vi "Resonance_Test.vi"(0 "Semiconductor Module Context":T7, 1 "FGEN Pin":T1, 2 "SCOPE Pins":T1[](array[typedef]), 3 "FGEN_Parameters":T2 {"Trigger Mode" items=["Single", "Continuous", "Stepped", "Burst"]}, 4 "SCOPE_Parameters":T4={"min sample rate"=20000000.0, "min record length"=1000, "reference position"=5.0, "input impedance"=0, "maximum input frequency"=0.0, "vertical coupling"=1, "vertical range"=10.0, "vertical offset"=0.0, "NumRecords"=0} {"maximum input frequency" format="%.2f"; "input impedance" items=["1 mega ohm"=0, "50 ohms"=2]; "vertical offset" format="%.4f"; "vertical range" format="%.2f"; "vertical coupling" items=["AC", "DC", "Ground"]; "reference position" format="%#_13g"; "min sample rate" format="%^.2e"}, 6 "Published Data Id":T6) -> (19 "error out":errorcluster)   [LabVIEW 2023, in "Resonance.lvlib"]
doc: "Configures SMU/AWG and start generating; if using SMU it also measures back the voltage applied.\nThe SCOPE acquires N channels and averages the samples of each channel.\nThe Offset is computed by dividing the average value with the applied voltage or Vrms of Sine wave when using AWG"
uses:
  Resonance.lvlib
  <vilib>/NI_TestStand_SemiconductorModule/NI_TestStand_Semiconductor_Module.lvlibp/PinMap/General/SemiconductorModuleContext.ctl
  <vilib>/NI_TestStand_SemiconductorModule/NI_TestStand_Semiconductor_Module.lvlibp/PinMap/TagProvider/TSM_Pin.ctl
  <vilib>/NI_TestStand_SemiconductorModule/NI_TestStand_Semiconductor_Module.lvlibp/PinMap/TagProvider/TSM_PublishedDataId.ctl
  ResourceHandling/TypeDefs/RH_SCOPE_Parameters.ctl
  <instrlib>/niScope/Controls/niScope vertical coupling.ctl
  ResourceHandling/TypeDefs/RH_FGEN_Parameters.ctl
  <instrlib>/niFgen/niFgen.llb/niFgen Trigger Mode.ctl
  <instrlib>/niFgen/niFgen.llb/niFgen_ctl Exported Signal Desination Values (ComboBox).ctl
  <instrlib>/niScope/Controls/niScope trigger source digital.ctl
  <vilib>/NI_TestStand_SemiconductorModule/NI_TestStand_Semiconductor_Module.lvlibp/PinMap/Scope/PinsToNISCOPESession.vi
  <vilib>/NI_TestStand_SemiconductorModule/NI_TestStand_Semiconductor_Module.lvlibp/PinMap/FGEN/PinToNIFGenSession.vi
  <instrlib>/niScope/Acquire/Fetch/niScope Multi Fetch WDT.vi
  <vilib>/NI_TestStand_SemiconductorModule/NI_TestStand_Semiconductor_Module.lvlibp/PinMap/General/Publish/PublishDataPerSiteDoubleScalar.vi
  ResourceHandling/ResourceHandling.lvlib
  <vilib>/NI_TestStand_SemiconductorModule/NI_TestStand_Semiconductor_Module.lvlibp
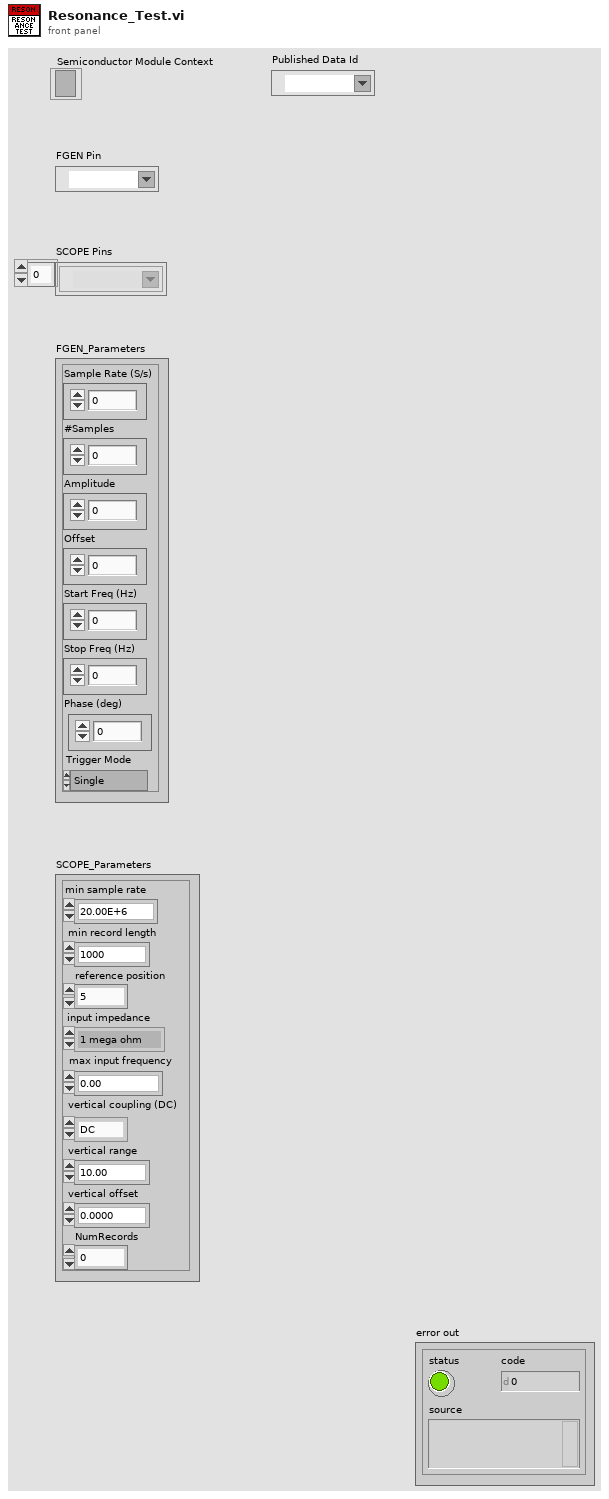
[diagram p1: front panel]
types:
  T1 = typedef "NI_TestStand_Semiconductor_Module.lvlibp/TSM_Pin.ctl" = tag
  T2 = typedef "ResourceHandling.lvlib/RH_FGEN_Parameters.ctl" = cluster{"Sample Rate (S/s)":dbl, "#Samples":i32, "Amplitude":dbl, "Offset":dbl, "Start Freq (Hz)":dbl, "Stop Freq (Hz)":dbl, "Phase (deg)":dbl, "Trigger Mode":T3}
  T3 = typedef "niFgen Trigger Mode.ctl" = i32
  T4 = typedef "ResourceHandling.lvlib/RH_SCOPE_Parameters.ctl" = cluster{"min sample rate":dbl, "min record length":i32, "reference position":dbl, "input impedance":u32, "maximum input frequency":dbl, "vertical coupling":T5, "vertical range":dbl, "vertical offset":dbl, "NumRecords":i32}
  T5 = typedef "niScope vertical coupling.ctl" = i32
  T6 = typedef "NI_TestStand_Semiconductor_Module.lvlibp/TSM_PublishedDataId.ctl" = tag
  T7 = typedef "NI_TestStand_Semiconductor_Module.lvlibp/SemiconductorModuleContext.ctl" = refnum<k7>
  T8 = typedef "niScope trigger source digital.ctl" = string
  T9 = typedef "niFgen_ctl Exported Signal Desination Values (ComboBox).ctl" = string
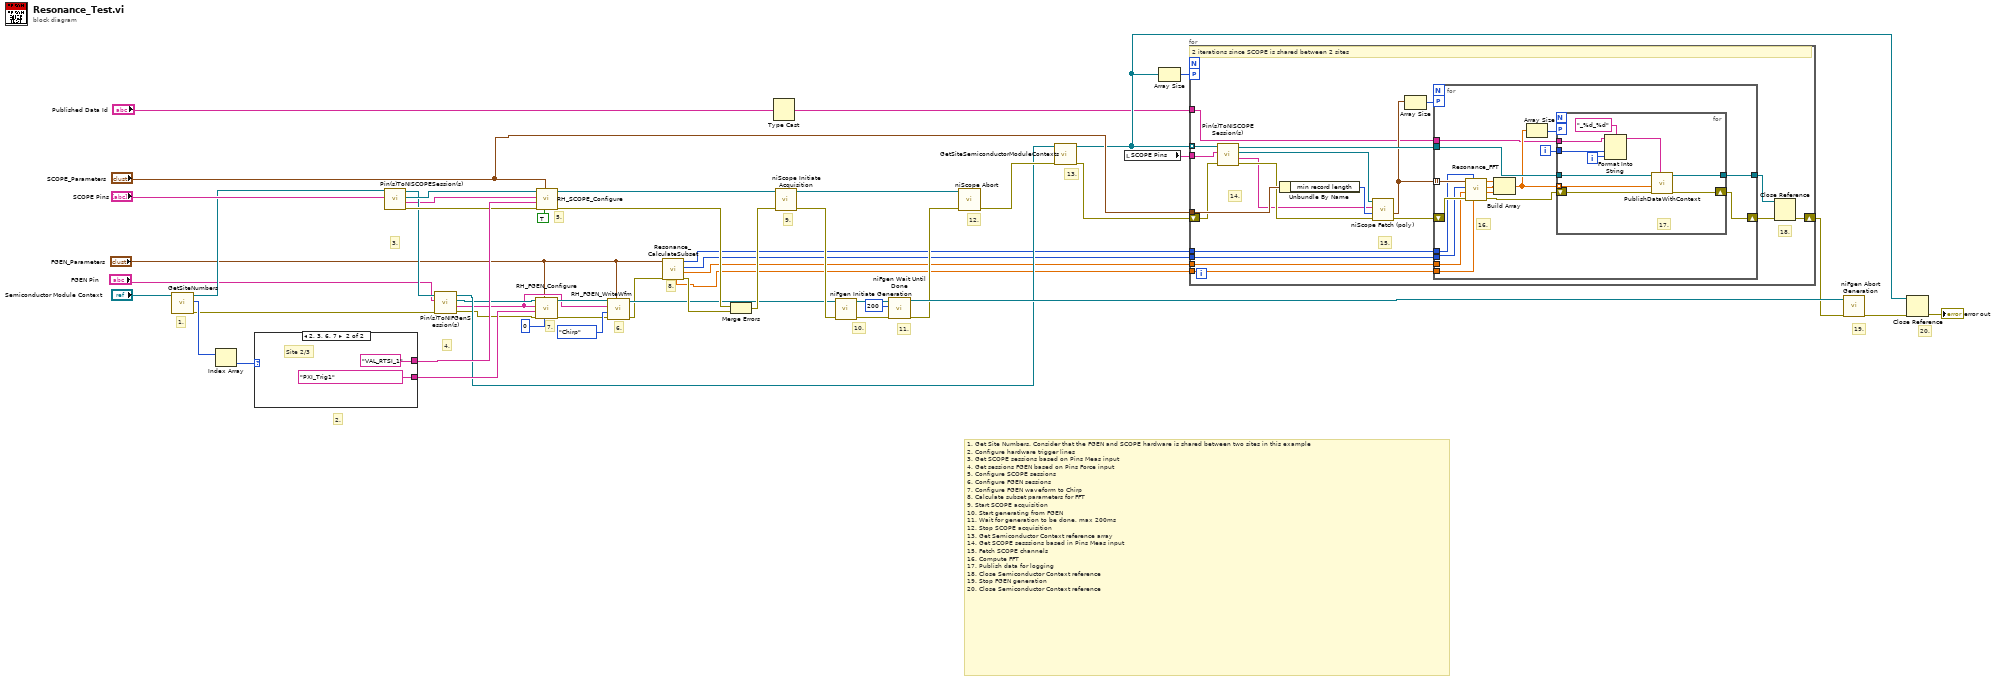
[diagram p0: block diagram]
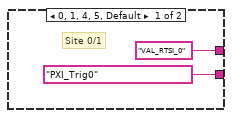
[diagram p2: hidden frame]
diagram:
  # "19."
  # "12."
  # "11."
  # "10."
  # "9."
  # "8."
  # "7."
  # "6."
  # "5."
  # "13."
  # "4."
  # "3."
  # "20."
  # "1. Get Site Numbers. Consider that the FGEN and SCOPE hardware is shared between two sites in this example\n2. Configure hardware trigger lines \n3. Get SCOPE sessions based on Pins Meas input\n4. Get sessions FGEN based on Pins Force input\n5. Configure SCOPE sessions\n6. Configure FGEN sessions\n7. Configure FGEN waveform to Chirp\n8. Calculate subset parameters for FFT\n9. Start SCOPE acquisition\n10. Start generating from FGEN\n11. Wait for generation to be done, max 200ms\n12. Stop SCOPE acquisition\n13. Get Semiconductor Context reference array\n14. Get SCOPE sesssions based in Pins Meas input\n15. Fetch SCOPE channels\n16. Compute FFT\n17. Publish data for logging\n18. Close Semiconductor Context reference\n19. Stop FGEN generation\n20. Close Semiconductor Context reference"
  # "2."
  # "1."
  n1 = call <vilib>:"GetSiteNumbers.vi"("Semiconductor Module Context"="Semiconductor Module Context") -> ("error out"=w33:errorcluster, "Site Numbers"=w47:i32[], "Semiconductor Module Context Out"=w44:T7)  [unwired: 7 in, 1 out]
  n2 = Index Array(array=w47) -> (element=w20:i32)  [unwired: 1 in]
  n3 = case shown="2, 3, 6, 7" w20 {
    tunnel: [T9 "PXI_Trig0" ("Output Terminal (do not export)") T9 "PXI_Trig1" ("Output Terminal (do not export)")] -> w46
    tunnel: [T8 "VAL_RTSI_0" ("trigger source") T8 "VAL_RTSI_1" ("trigger source")] -> w45
    frame 0, 1, 4, 5, Default {
      # "Site 0/1"
    }
    frame 2, 3, 6, 7 {
      # "Site 2/3"
    }
  }
  n4 = call-poly <vilib>:"Pin(s)ToNISCOPESession(s).vi"("Pins"="SCOPE Pins", "Semiconductor Module Context"=w44) -> ("error out"=w42:errorcluster, "Channel List"=w34:string, "Instrument Session"=w43:refnum<k15>, "Semiconductor Module Context Out"=w41:T7)  [unwired: 5 in, 1 out]
  n5 = call-poly <vilib>:"Pin(s)ToNIFGenSession(s).vi"("error in (no error)"=w33, "Pin"="FGEN Pin", "Semiconductor Module Context"=w41) -> ("error out"=w7:errorcluster, "Channel List"=w2:string, "Instrument Session"=w8:refnum<k15>, "Semiconductor Module Context Out"=w29:T7)  [unwired: 4 in, 1 out]
  n6 = call "RH_FGEN_Configure.vi"("Marker Position"=0, "FGEN Parameters"="FGEN_Parameters", "error in"=w7, "Output Terminal (do not export)"=w46, "Channel Name"=w2, "FGEN Session In"=w8) -> ("error out"=w5:errorcluster, "FGEN Session Out"=w6:refnum<k15>)  [unwired: 4 in]
  n7 = call "RH_SCOPE_Configure.vi"("Digital Trigger?"=TRUE, "SCOPE Global Parameters"="SCOPE_Parameters", "error in"=w42, "trigger source"=w45, "channels"=w34, "SCOPE Session In"=w43) -> ("error out"=w39:errorcluster, "SCOPE Session Out"=w38:refnum<k15>)  [unwired: 4 in]
  n8 = call "RH_FGEN_WriteWfm.vi"("FGEN Parameters"="FGEN_Parameters", "error IO"=w5, "Wfm Type"=enum16{"Chirp", "MultiSine", "Sine"}."Chirp", "Channel Name"=w2, "FGEN Session In"=w6) -> ("error out"=w3:errorcluster, "FGEN Session Out"=w4:refnum<k15>)  [unwired: 5 in]
  n9 = call "Resonance_CalculateSubset.vi"("error in"=w3, "FGEN Parameters"="FGEN_Parameters") -> ("error out"=w40:errorcluster, "dF"=w22:dbl, "Length"=w23:i32, "Index"=w24:i32, "Start Offset"=w21:dbl)  [unwired: 5 in]
  n10 = Merge Errors(w39, w40) -> (w37:errorcluster)
  n11 = Type Cast(x="Published Data Id") -> (*(type *) &x=w9:string)  [unwired: 1 in]
  n12 = call <instrlib>:"niScope Initiate Acquisition.vi"("instrument handle"=w38, "error in"=w37) -> ("instrument handle out"=w32:refnum<k15>, "error out"=w36:errorcluster)  [unwired: 12 in]
  n13 = call <instrlib>:"niFgen Initiate Generation.vi"("error in (no error)"=w36, "Instrument Handle"=w4) -> ("error out"=w12:errorcluster, "Instrument Handle Out"=w11:refnum<k15>)  [unwired: 8 in]
  n14 = call <instrlib>:"niFgen Wait Until Done.vi"("error in (no error)"=w12, "MaxTime (msec)"=200, "Instrument Handle"=w11) -> ("error out"=w31:errorcluster, "Instrument Handle Out"=w35:refnum<k15>)  [unwired: 7 in]
  n15 = call <instrlib>:"niScope Abort.vi"("instrument handle"=w32, "error in"=w31) -> ("error out"=w30:errorcluster)  [unwired: 12 in, 1 out]
  n16 = call <vilib>:"GetSiteSemiconductorModuleContexts.vi"("error in (no error)"=w30, "Semiconductor Module Context"=w29) -> ("error out"=w28:errorcluster, "Site Semiconductor Module Contexts"=w17:T7[])  [unwired: 8 in]
  n17 = local read "SCOPE Pins"() -> (w26:T1[])
  n18 = Array Size(array=w17) -> (size(s)=w25:i32)
  n19 = for {
    shift-right: [w56] -> w19
    shift-left: w28 -> [w72]
    tunnel: "SCOPE_Parameters" -> [w75]
    tunnel: w17 -> [w73] mode=indexing
    tunnel: w26 -> [w71]
    workers-P: w25 -> [_]
    tunnel: w24 -> [w65]
    tunnel: w23 -> [w64]
    tunnel: w22 -> [w63]
    tunnel: w21 -> [w62]
    tunnel: w9 -> [w59]
    # "18."
    # "15."
    # "14."
    # "2 iterations since SCOPE is shared between 2 sites"
    n20 = call-poly <vilib>:"Pin(s)ToNISCOPESession(s).vi"("error in (no error)"=w72, "Pins"=w71, "Semiconductor Module Context"=w73) -> ("error out"=w70:errorcluster, "Channel List"=w68:string, "Instrument Session"=w69:refnum<k15>, "Semiconductor Module Context Out"=w66:T7)  [unwired: 4 in, 1 out]
    n21 = Unbundle By Name(w75) -> ("min record length"=w74:i32)
    n22 = call-poly <instrlib>:"niScope Fetch (poly).vi"("error in"=w70, "numSamples"=w74, "channels"=w68, "instrument handle"=w69) -> ("error out"=w67:errorcluster, "wfm"=w60:waveform(dbl)[])  [unwired: 4 in, 2 out]
    n23 = Array Size(array=w60) -> (size(s)=w61:i32)
    n24 = for {
      tunnel: w60 -> [w87] mode=indexing
      tunnel: w66 -> [w85]
      tunnel: w65 -> [w83]
      tunnel: w64 -> [w82]
      tunnel: w63 -> [w81]
      tunnel: w62 -> [w84]
      shift-right: [w77] -> w58
      shift-left: w67 -> [w89]
      workers-P: w61 -> [_]
      tunnel: w59 -> [w78]
      tunnel: [w76] -> w57
      i -> [w86]
      # "16."
      n25 = call "Resonance_FFT.vi"("Start Offset"=w84, "Index"=w83, "error in"=w89, "dF"=w81, "Length"=w82, "Waveform"=w87) -> ("error out"=w88:errorcluster, "Phase"=w92:dbl, "Frequency"=w91:dbl, "Amplitude"=w90:dbl)  [unwired: 2 in]
      n26 = Build Array(w90, w91, w92) -> (w79:dbl[])
      n27 = Array Size(array=w79) -> (size(s)=w80:i32)
      n28 = for {
        shift-right: [w98] -> w77
        shift-left: w88 -> [w102]
        tunnel: w79 -> [w96] mode=indexing
        tunnel: w86 -> [w94]
        workers-P: w80 -> [_]
        tunnel: w85 -> [w101]
        tunnel: [w97] -> w76
        tunnel: w78 -> [w93]
        i -> [w95]
        # "17."
        n29 = Format Into String(format string="_%d_%d", initial string=w93, w94, w95) -> (resulting string=w99:string)  [unwired: 1 in, 1 out]
        n30 = call-poly <vilib>:"PublishDataWithContext.vi"("Published Data Id"=w99, "error in (no error)"=w102, "Data In"=w96, "Semiconductor Module Context"=w101) -> ("error out"=w98:errorcluster, "Semiconductor Module Context Out"=w97:T7)  [unwired: 6 in]
      }
    }
    n31 = Close Reference(reference=w57, error in (no error)=w58) -> (error out=w56:errorcluster)
  }
  n32 = call <instrlib>:"niFgen Abort Generation.vi"("error in (no error)"=w19, "Instrument Handle"=w35) -> ("error out"=w18:errorcluster)  [unwired: 8 in, 1 out]
  n33 = Close Reference(reference=w17, error in (no error)=w18) -> (error out=→"error out":errorcluster)
